vi "Preconditioning.vi"(8 "error in":errorcluster, 10 "Sequence Context":refnum<k7>, 11 "PreUUT":refnum<class "PreUUT.lvclass">=refnum) -> (0 "error out":errorcluster, 2 "Preconditioning":bool, 3 "PreUUT out":refnum<class "PreUUT.lvclass">)   [LabVIEW 2025, in "PreUUT.lvclass"]
uses:
  PreUUT.lvclass
  C:/Working copy/TS Manager/Plugin/Tests/Submodule EOL/TS Execution Interface/OPC UA/Abstract.lvclass
  OPC UA/Read Rx from PLC.vi
  <vilib>/addons/TestStand/_TSUtility.llb/TestStand - Get Property Value (String).vi
  <vilib>/addons/TestStand/_TSUtility.llb/TestStand - Set Property Value (String).vi
  <vilib>/addons/TestStand/_TSUtility.llb/TestStand - Set Property Value (Number {Signed 32-bit Integer}).vi
  <vilib>/regexp/Match Regular Expression.xnode
panel:
  out "PN_SN":string="P:10-000001R:04S:QMC2200123"
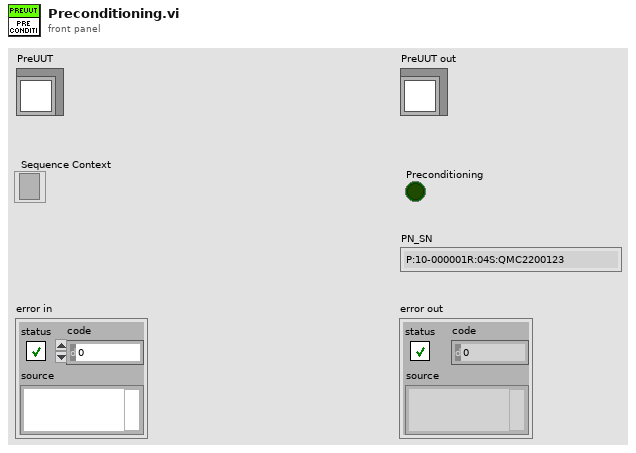
[diagram p1: front panel]
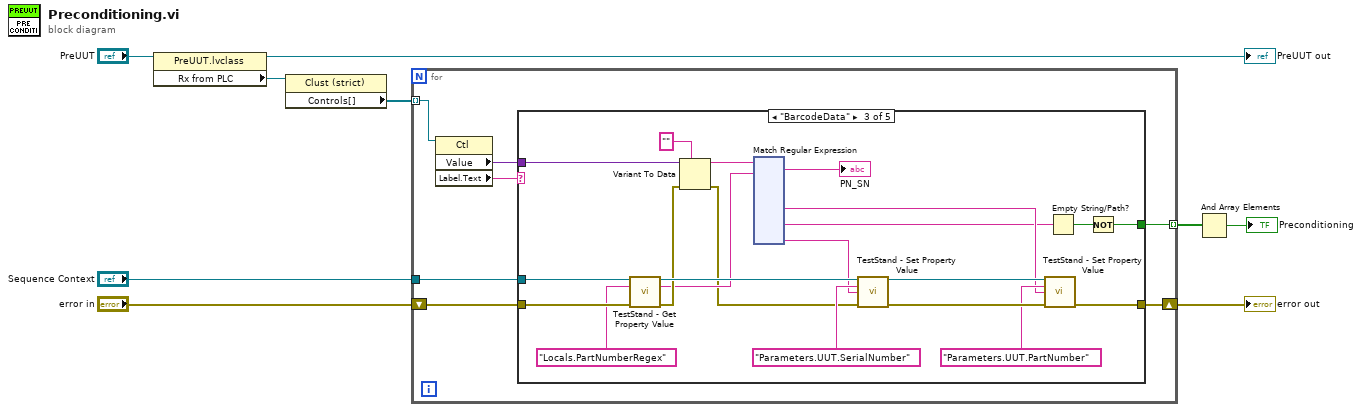
[diagram p0: block diagram]
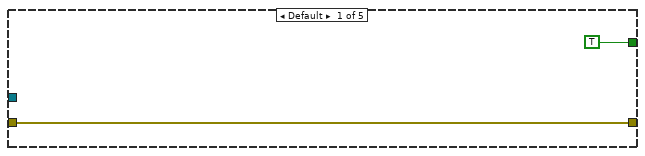
[diagram p2: hidden frame]
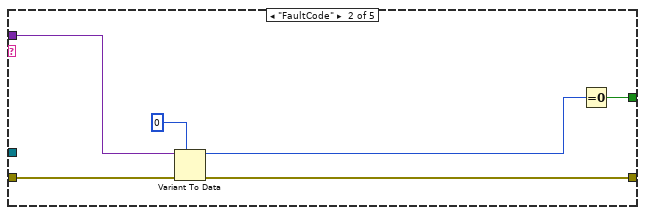
[diagram p3: hidden frame]
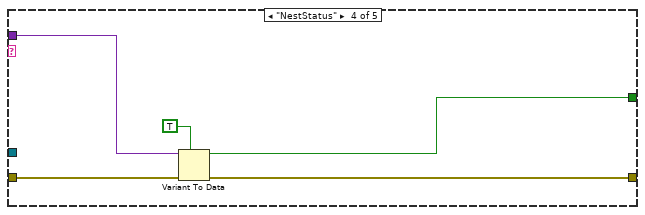
[diagram p4: hidden frame]
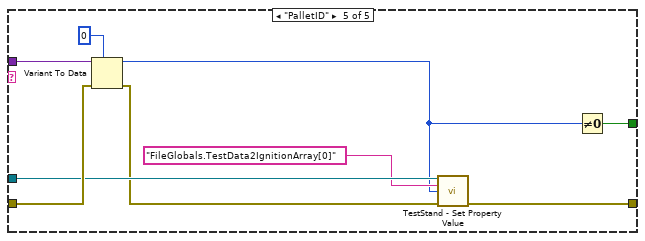
[diagram p5: hidden frame]
diagram:
  n1 = property class="PreUUT.lvclass"(reference="PreUUT") -> (reference out=→"PreUUT out":refnum<class "PreUUT.lvclass">, "Rx from PLC"=w1:refnum<vi>)  [unwired: 1 in, 1 out]
  n2 = property class="Clust (strict)"(reference=w1) -> ("Controls[]"=w2:refnum<vi>[])  [unwired: 1 in, 2 out]
  n3 = for {
    tunnel: w2 -> [w16] mode=indexing
    shift-right: [w14] -> w8
    shift-left: "error in" -> [w15]
    tunnel: "Sequence Context" -> [w13]
    tunnel: [w12] -> w3 mode=indexing
    n4 = property class="Ctl"(reference=w16) -> ("Value"=w10:variant, "Label.Text"=w11:string)  [unwired: 1 in, 2 out]
    n5 = case shown="\"BarcodeData\"" w11 {
      tunnel: w10 -> [_ w23 w45 w172 w182]
      tunnel: [TRUE w19 w37 w171 w180] -> w12
      tunnel: w15 -> [w18 w24 w36 w173 w183]
      tunnel: [w18 w22 w41 w170 w176] -> w14
      tunnel: w13 -> [_ _ w35 _ w179]
      frame Default {
      }
      frame "FaultCode" {
        n6 = Variant To Data(error in=w24, type=0, Variant=w23) -> (data=w20:i32, error out=w22:errorcluster)
        n7 = Equal To 0?(x=w20) -> (x = 0?=w19:bool)
      }
      frame "BarcodeData" {
        n8 = call-poly <vilib>:"TestStand - Get Property Value.vi"("Sequence Context In"=w35, "Lookup String"="Locals.PartNumberRegex", "error in (no error)"=w36) -> ("Sequence Context Out"=w34:refnum<k7>, "Value"=w31:string, "error out"=w32:errorcluster)  [unwired: 10 in]
        n9 = Variant To Data(error in=w32, type="", Variant=w45) -> (data=w30:string, error out=w29:errorcluster)
        n10 = xnode "Match Regular Expression"("input string"=w30, "regular expression"=w31) -> ("whole match"=→"PN_SN":string, "submatch 2"=w27:string, "submatch 4"=w26:string, "submatch 6"=w28:string)  [unwired: 4 in, 7 out]
        n11 = call-poly <vilib>:"TestStand - Set Property Value.vi"("Sequence Context In"=w34, "Lookup String"="Parameters.UUT.SerialNumber", "New Value"=w28, "error in (no error)"=w29) -> ("Sequence Context Out"=w39:refnum<k7>, "error out"=w42:errorcluster)  [unwired: 10 in]
        n12 = call-poly <vilib>:"TestStand - Set Property Value.vi"("Sequence Context In"=w39, "Lookup String"="Parameters.UUT.PartNumber", "New Value"=w27, "error in (no error)"=w42) -> ("error out"=w41:errorcluster)  [unwired: 10 in, 1 out]
        n13 = Empty String/Path?(string/path=w26) -> (empty?=w38:bool)
        n14 = Not(x=w38) -> (.not. x?=w37:bool)
      }
      frame "NestStatus" {
        n15 = Variant To Data(error in=w173, type=TRUE, Variant=w172) -> (data=w171:bool, error out=w170:errorcluster)
      }
      frame "PalletID" {
        n16 = Variant To Data(error in=w183, type=0, Variant=w182) -> (data=w175:i32, error out=w177:errorcluster)
        n17 = call-poly <vilib>:"TestStand - Set Property Value.vi"("Sequence Context In"=w179, "Lookup String"="FileGlobals.TestData2IgnitionArray[0]", "New Value"=w175, "error in (no error)"=w177) -> ("error out"=w176:errorcluster)  [unwired: 10 in, 1 out]
        n18 = Not Equal To 0?(x=w175) -> (x != 0?=w180:bool)
      }
    }
  }
  "error out" <- w8
  n19 = And Array Elements(Boolean array=w3) -> (logical AND=→"Preconditioning":bool)
